vi "ScreenMenu.vi"(0 "ip":string) -> ()   [LabVIEW 2024]
panel:
  in  "Percentage":dbl(slide) step=1.0 scale=0.0..100.0 scale format="%#.6g"
  in  "Voltage":dbl(slide) step=1.0 scale=0.0..510.0
  in  "Cancel Button":bool
  in  "OK Button":bool
  # "OLED Screen Setting Menu"
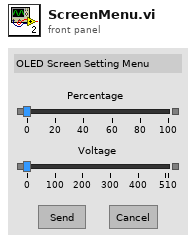
[diagram p1: front panel]
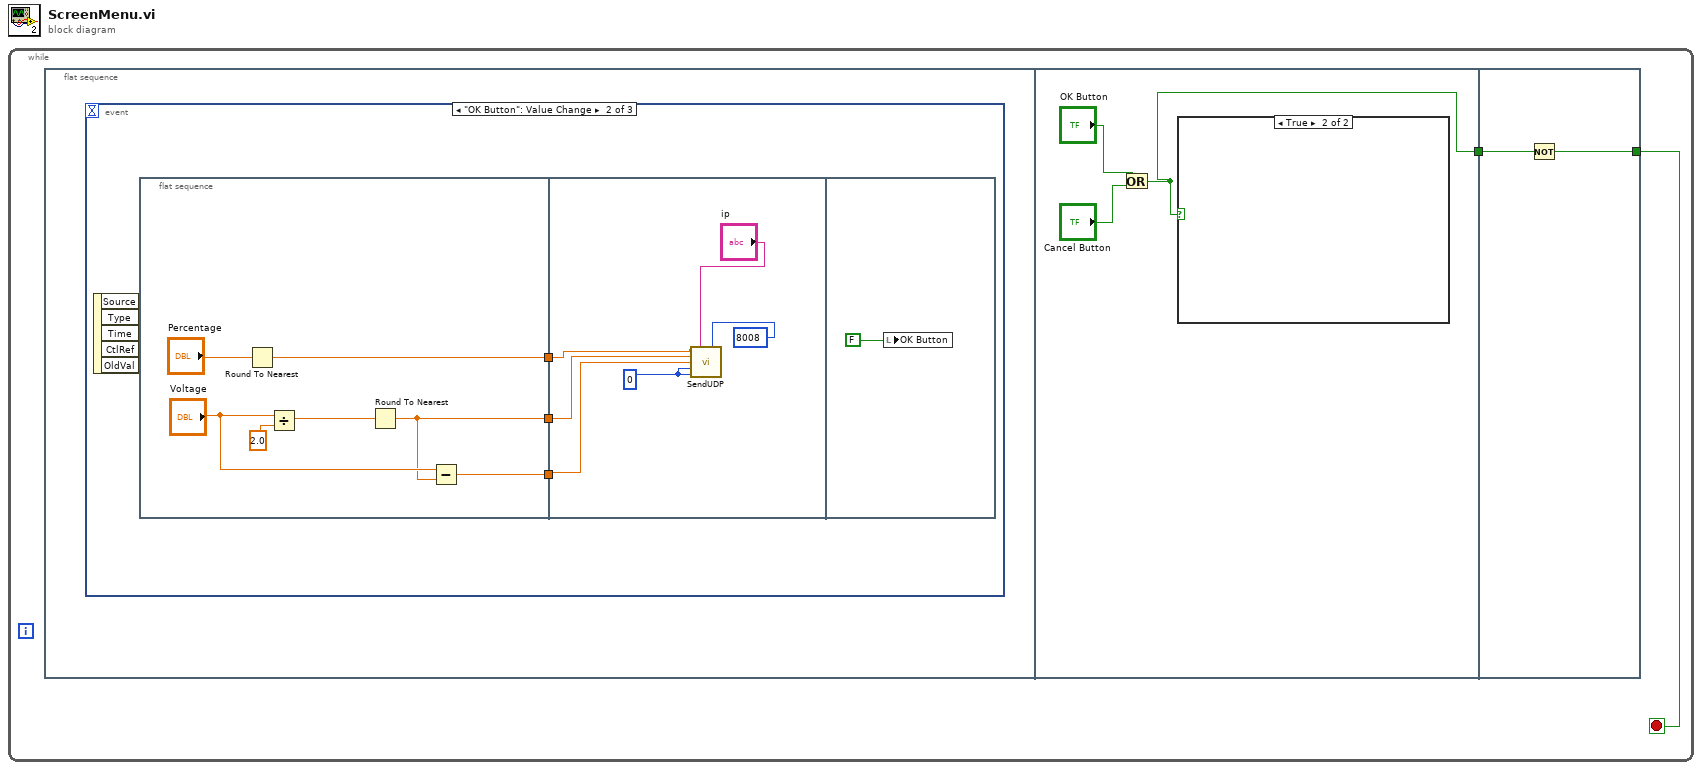
[diagram p0: block diagram]
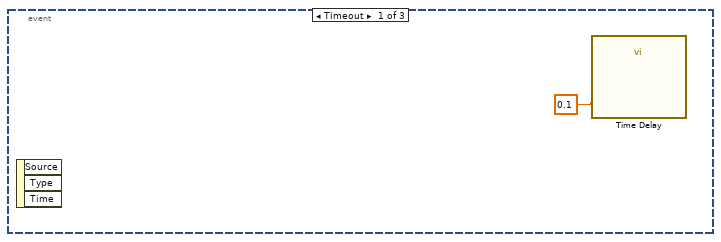
[diagram p2: hidden frame]
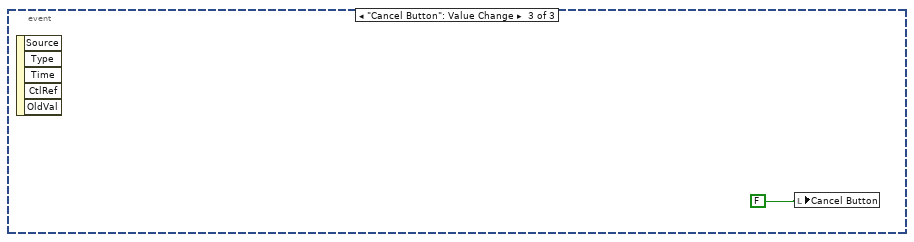
[diagram p3: hidden frame]
diagram:
  n1 = while {
    stop <- w2 stop-if-true
    n2 = flat-sequence {
      tunnel: [w22] -> w1
      tunnel: [w26] -> w2
      tunnel: w1 -> [w25]
      frame #0 {
        n3 = event shown="[1] \"OK Button\": Value Change" {
          selector: _ -> [_ _ _]
          dyn-events: _ -> [_ _ _]
          timeout: _ -> [_ _ _]
          event Timeout {
            n4 = event-data() -> ()  [unwired: 1 in, 3 out]
            n5 = call "Time Delay"("Delay Time (s)"=0.1) -> ()  [unwired: 10 in, 1 out]
          }
          event "OK Button": Value Change {
            n6 = event-data() -> ()  [unwired: 1 in, 5 out]
            n7 = flat-sequence {
              tunnel: [w12] -> w6
              tunnel: [w8] -> w5
              tunnel: [w7] -> w4
              tunnel: w6 -> [w17]
              tunnel: w5 -> [w16]
              tunnel: w4 -> [w15]
              frame #0 {
                n8 = Round To Nearest(number="Percentage") -> (nearest integer value=w12:dbl)
                n9 = Divide(x="Voltage", y=2.0) -> (x/y=w11:dbl)
                n10 = Round To Nearest(number=w11) -> (nearest integer value=w8:dbl)
                n11 = Subtract(x="Voltage", y=w8) -> (x-y=w7:dbl)
              }
              frame #1 {
                w14 = u8 0 ("Arg7")
                n12 = call "SendUDP.vi"("Arg3"=w17, "IP"="ip", "Port"=8008, "Arg4"=w16, "Arg5"=w15, "Arg6"=w14, "Arg7"=w14) -> ()  [unwired: 9 in]
              }
              frame #2 {
                n13 = local write "OK Button"(FALSE ("OK Button")) -> ()
              }
            }
          }
          event "Cancel Button": Value Change {
            n14 = event-data() -> ()  [unwired: 1 in, 5 out]
            n15 = local write "Cancel Button"(FALSE ("Cancel Button")) -> ()
          }
        }
      }
      frame #1 {
        n16 = Or(x="OK Button", y="Cancel Button") -> (x .or. y?=w22:bool)
        n17 = case shown="True" w22 {
          frame False {
          }
          frame True {
          }
        }
      }
      frame #2 {
        n18 = Not(x=w25) -> (.not. x?=w26:bool)
      }
    }
  }
